vi "AutoOp Default.vi"(10 "Occurrence Refnum":refnum<k4>, 11 "OpMode Index":u64 format="%.0x") -> ()   [LabVIEW 2023]
uses:
  <vilib>/MRC/MrcLib.lvlib
panel:
  out "Enabled":bool
  out "Match Time(s)":sgl
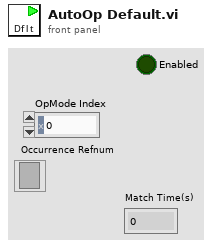
[diagram p1: front panel]
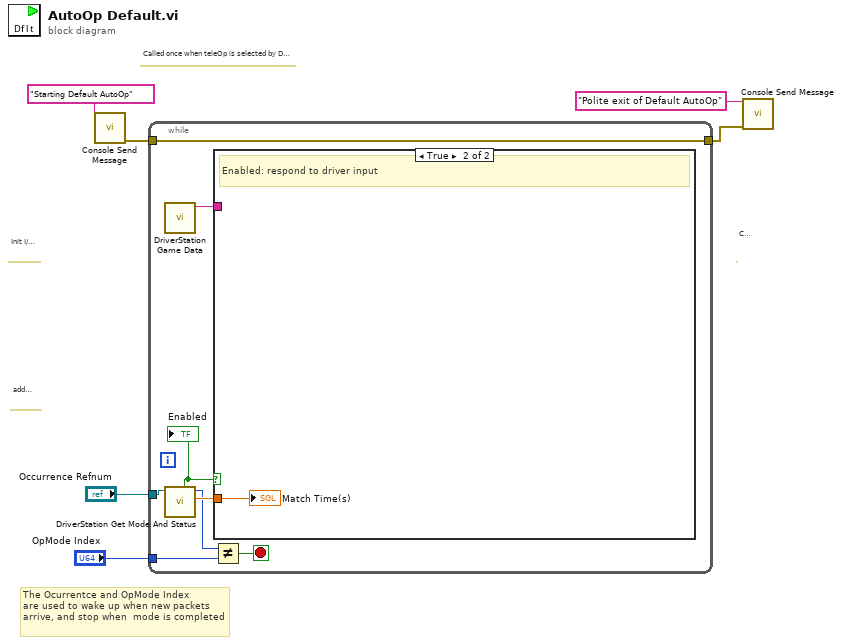
[diagram p0: block diagram]
diagram:
  # "The Ocurrentce and OpMode Index\nare used to wake up when new packets\narrive, and stop when  mode is completed"
  # "add enabled counter\nstats, etc"
  # "Cleanup I/O"
  # "Called once when teleOp is selected by DS.\nLoop until mode changes carrying out enabled\nor disabled response."
  # "Init I/O and anything\nused during TeleOp"
  n1 = call <vilib>:"Console Send Message.vi"("Message"="Starting Default AutoOp") -> ("error out"=w4:errorcluster)  [unwired: 14 in]
  n2 = while {
    tunnel: "OpMode Index" -> [w13]
    tunnel: w4 -> [w10]
    tunnel: [w10] -> w2
    tunnel: "Occurrence Refnum" -> [w9]
    stop <- w12 stop-if-true
    n3 = call <vilib>:"DriverStation Game Data.vi"() -> ("Game Specific Data"=w7:string)  [unwired: 11 in]
    n4 = call <vilib>:"DriverStation Get Mode And Status.vi"("Occurrence Refnum"=w9) -> ("Match Time(s)"=w14:sgl, "currentOpMode"=w11:u64, "Enabled"=w8:bool)  [unwired: 5 in, 3 out]
    "Enabled" <- w8
    n5 = Not Equal?(x=w11, y=w13) -> (x != y?=w12:bool)
    n6 = case shown="True" w8 {
      tunnel: w14 -> [_ w15]
      tunnel: w7 -> [_ _]
      frame False {
        # "Disabled: update dashboard, possibly update state and setpoints for a safer enable"
      }
      frame True {
        # "Enabled: respond to driver input"
        "Match Time(s)" <- w15
      }
    }
  }
  n7 = call <vilib>:"Console Send Message.vi"("Message"="Polite exit of Default AutoOp", "error in (no error)"=w2) -> ()  [unwired: 13 in, 1 out]
